vi "Native_AddInputChunk.vi"() -> ()   [LabVIEW 2024]
panel:
  out "error out":errorcluster caption="错误输出"
  out "terminal_ids":u32[](array[numeric])
  in  "terminal_ids type":u32
  in  "chunks":u8
  in  "object_id":u32
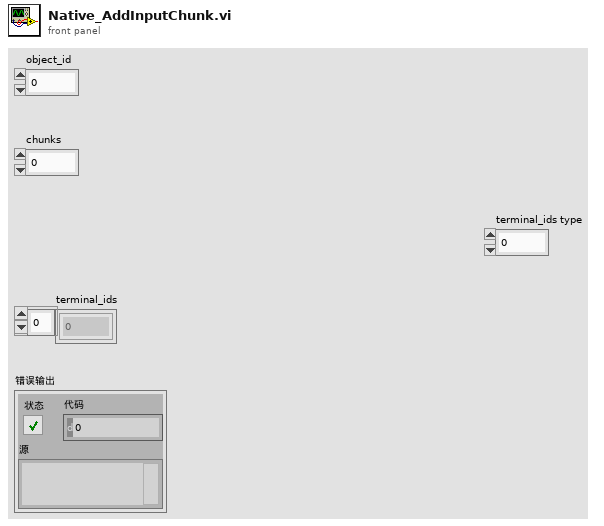
[diagram p1: front panel]
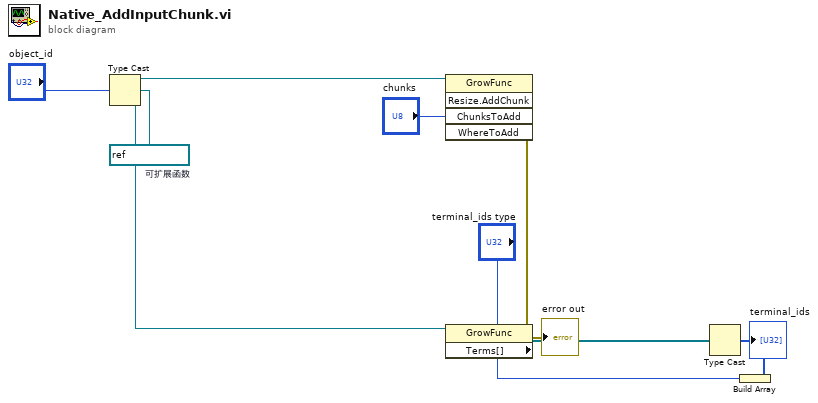
[diagram p0: block diagram]
diagram:
  w9 = refnum<vi> refnum  # 可扩展函数
  n1 = Type Cast ("强制类型转换")(type=w9, x="object_id") -> (*(type *) &x=w8:refnum<vi>)
  n2 = invoke class="GrowFunc" method="Resize.AddChunk"(reference=w8, "ChunksToAdd"="chunks") -> (error out=w6:errorcluster)  [unwired: 3 in, 4 out]
  n3 = property on="属性节点" class="GrowFunc"(reference=w8, error in=w6) -> (error out=→"error out":errorcluster, "Terms[]"=w5:refnum<vi>[])  [unwired: 1 out]
  n4 = Build Array ("创建数组")("terminal_ids type") -> (w3:u32[])
  n5 = Type Cast ("强制类型转换")(type=w3, x=w5) -> (*(type *) &x=→"terminal_ids":u32[])
